vi "Tx.vi"() -> ()   [LabVIEW 2025]
uses:
  <vilib>/sound2/lvsound2.llb/Sound File Position.ctl
  <vilib>/addons/Modulation/Analog/support/mod_Set Error Source.vi
  <vilib>/addons/Modulation/Digital/General/MT Generate PSK System Parameters(M).vi
  <vilib>/addons/Modulation/Digital/Support/Common/Validators/mod_Generate Filter Coefficients Validate.vi
  <vilib>/addons/Modulation/Digital/General/subVIs/mod_Generate Filter Coefficients.vi
  <instrlib>/niUSRP/niUSRP Write Tx Data (CDB).vi
  <vilib>/addons/Modulation/niDMT.lvlib
panel:
  out "IQ Rate (actual)":dbl format="%#_6p"
  out "Carrier Frequency (actucal)":dbl=100000.0 format="%#_6p"
  out "Gain":dbl format="%#_6f"
  in  "modulation type":T1(ring)=enum."PSK"
  out "XY Graph 4":T2(graph)
  out "XY Graph 3":cdb[](graph)
  in  "PSK type":u16(ring) items=["normal", "shifted", "offset"]
  in  "M-PSK (4)":i32=8
  in  "differential PSK":enum16{"disable", "enable"}(ring)
  in  "filter parameter":dbl=0.8 format="%.2f"
  out "symbols out":cdb[](array[numeric]) format="%.2f"
  in  "error in":errorcluster
  out "size(s)":i32
  in  "error in (no error)":errorcluster
  out "error out":errorcluster
  in  "stop":bool
  out "BB Modulate":cluster{"t0":dbl, "dt":dbl, "Y":dbl[]}(graph)
  out "input":i16[](graph)
  in  "active antenna":string="TX1"
  in  "carrier frequency":dbl=2400000000.0 format="%#_6p"
  in  "gain":dbl format="%#_6f"
  in  "IQ rate":dbl=200000.0 format="%#_6p"
  in  "channel list":string
  in  "device names":refnum<k15>="NI2900"
  in  "filter length (symbols)":i32=8
  in  "symbol rate (Hz)":dbl=127500.0 format="%.2f"
  in  "samples per symbol (16)":i32=16
  in  "pulse shaping samples per symbol (16)":i32=16
  in  "pulse shaping filter (none)":T3(ring)=enum."Root Raised Cos"
  in  "number of samples/ch (-1: all)":i32=-1
  in  "start path":path=path ""
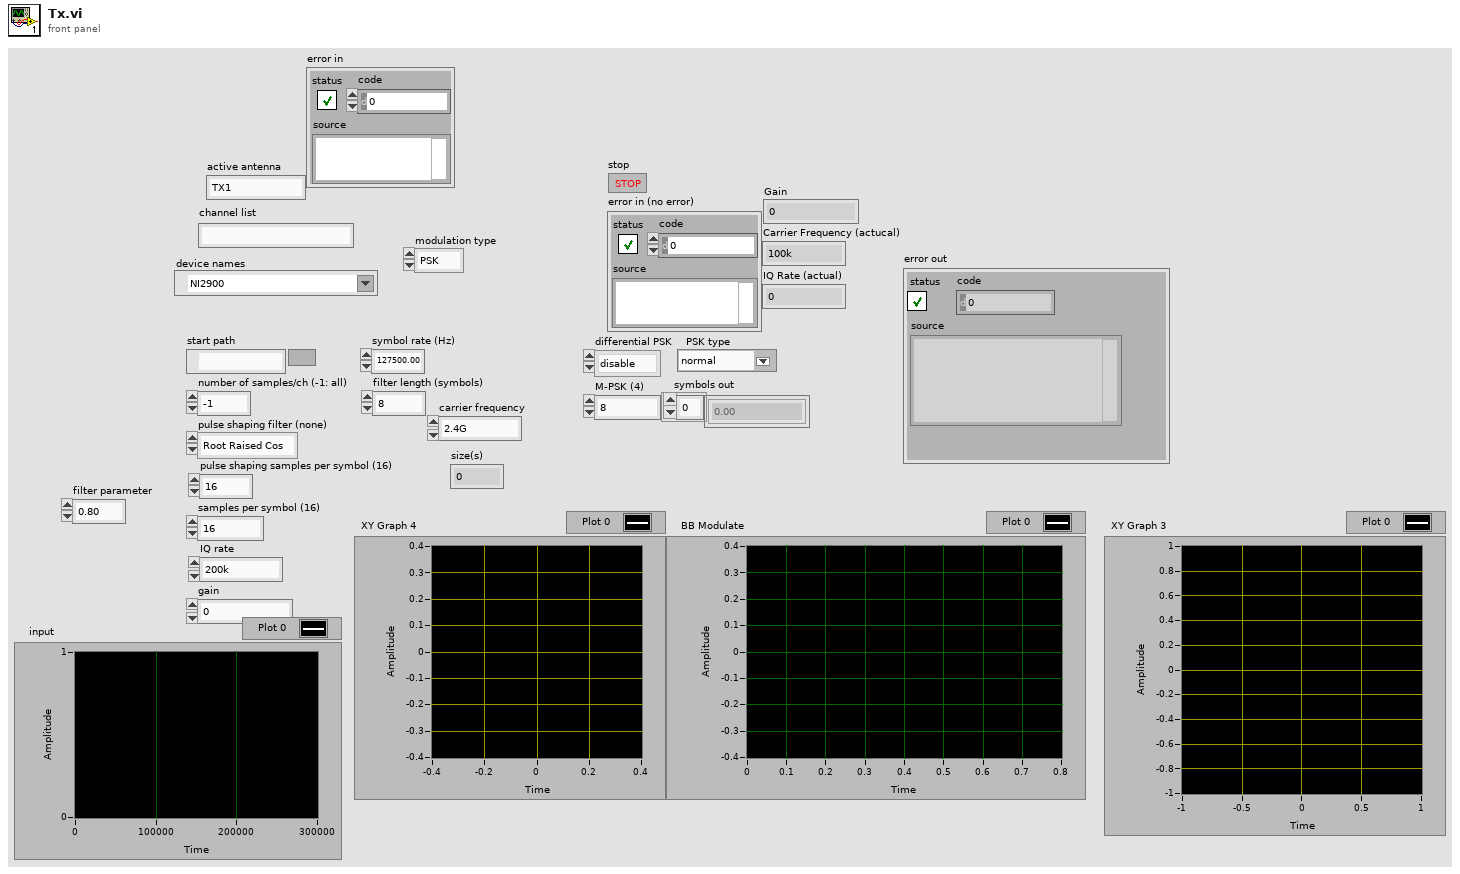
[diagram p1: front panel]
types:
  T1 = enum16{"FSK", "PSK", "QAM", "MSK", "PAM", "ASK", "CPM"}
  T2 = cluster{"constellation":dbl[], "oversampled data":dbl[]}[]
  T3 = enum16{"none", "Raised Cosine", "Root Raised Cos", "Gaussian"}
  T4 = typedef "Sound File Position.ctl" = u16
  T5 = cluster{"samples per symbol (16)":i32, "symbol map":cdb[], "differential PSK":enum16{"disable", "enable"}, "PSK type":u16}
  T6 = typedef "niAMT.lvlib/Complex Data Waveform.ctl" = cluster{"t0":dbl, "dt":dbl, "Y":cdb[]}
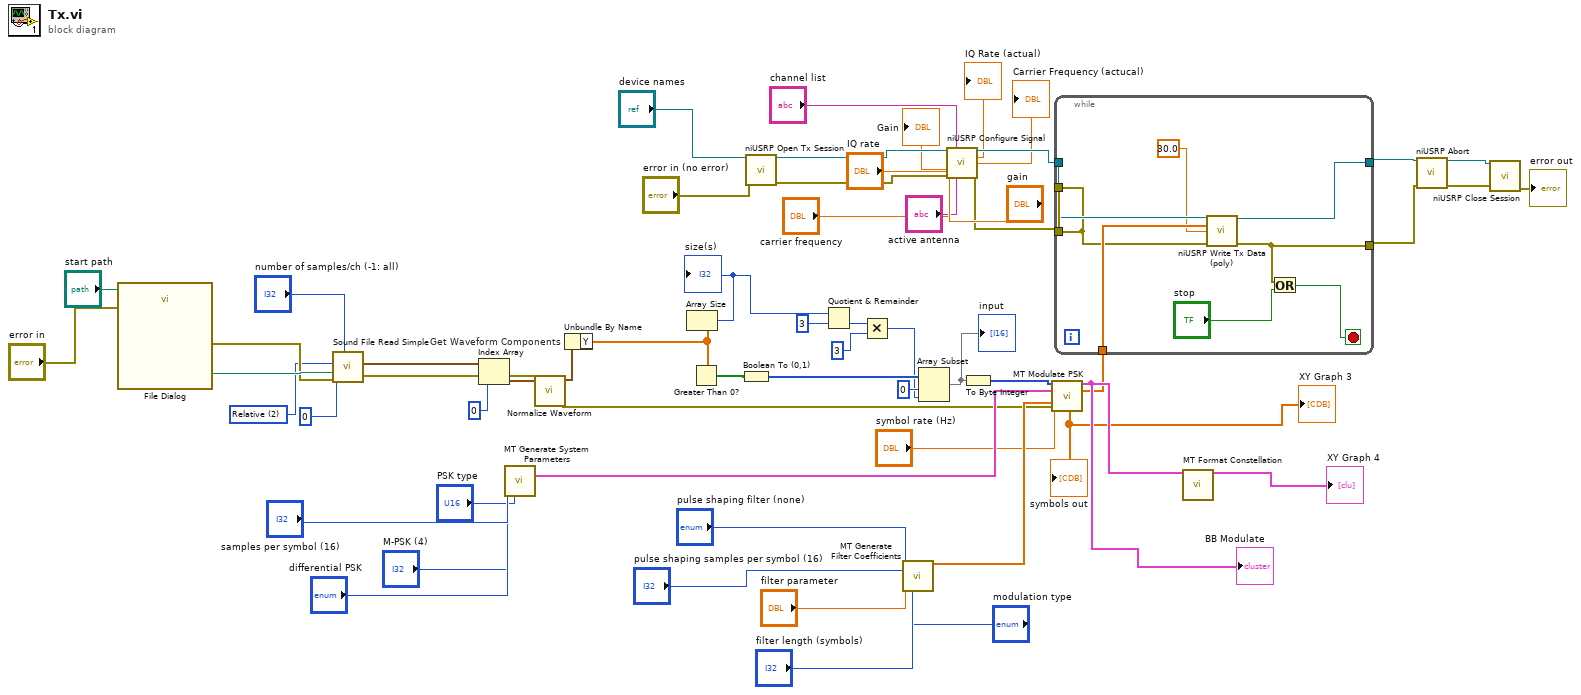
[diagram p0: block diagram]
diagram:
  w14 = T4 2 items=["Absolute"=0, "Relative"=2] ("position mode")
  n1 = call "File Dialog"("start path"="start path", "error in"="error in") -> ("selected path"=w57:path, "error out"=w27:errorcluster)  [unwired: 10 in, 2 out]
  n2 = call <vilib>:"Sound File Read Simple.vi"("number of samples/ch (-1: all)"="number of samples/ch (-1: all)", "error in (no error)"=w27, "position offset"=0, "position mode"=w14, "path"=w57) -> ("error out"=w26:errorcluster, "data"=w56:waveform(dbl)[])  [unwired: 3 in, 2 out]
  n3 = Index Array "Index Array"(array=w56, index=0) -> (element=w52:waveform(dbl))
  n4 = call-poly <vilib>:"MT Generate System Parameters.vi"("samples per symbol (16)"="samples per symbol (16)", "PSK type"="PSK type", "M-PSK (4)"="M-PSK (4)", "differential PSK"="differential PSK") -> ("PSK system parameters"=w40:T5)  [unwired: 9 in, 2 out]
  n5 = call <vilib>:"Normalize Waveform.vi"("error in (no error)"=w26, "waveform in"=w52) -> ("error out"=w25:errorcluster, "normalized waveform"=w51:waveform(dbl))  [unwired: 6 in, 2 out]
  n6 = Unbundle By Name "Get Waveform Components"(w51) -> ("Y"=w48:dbl[])
  n7 = Array Size(array=w48) -> (size(s)=w47:i32)
  "size(s)" <- w47
  n8 = Greater Than 0?(x=w48) -> (x > 0?=w50:bool[])
  n9 = Boolean To (0,1)(Boolean=w50) -> (0, 1=w49:i16[])
  n10 = call <instrlib>:"niUSRP Open Tx Session.vi"("device names"="device names", "error in (no error)"="error in (no error)") -> ("session handle out"=w37:refnum<k15>, "error out"=w24:errorcluster)  [unwired: 12 in]
  n11 = Quotient & Remainder(x=w47, y=3) -> (floor(x/y)=w13:i32)  [unwired: 1 out]
  n12 = Multiply(x=w13, y=3) -> (x*y=w45:i32)
  n13 = call <vilib>:"MT Generate Filter Coefficients.vi"("pulse shaping filter (none)"="pulse shaping filter (none)", "modulation type"="modulation type", "pulse shaping samples per symbol (16)"="pulse shaping samples per symbol (16)", "filter parameter"="filter parameter", "filter length (symbols)"="filter length (symbols)") -> ("pulse shaping filter coefficients"=w42:dbl[])  [unwired: 8 in, 2 out]
  n14 = Array Subset "Array Subset"(array=w49, index=0, length=w45) -> (w2:i16[])
  "input" <- w2
  n15 = call <instrlib>:"niUSRP Configure Signal.vi"("session handle"=w37, "channel list"="channel list", "IQ rate"="IQ rate", "carrier frequency"="carrier frequency", "gain"="gain", "error in (no error)"=w24, "active antenna"="active antenna") -> ("session handle out"=w16:refnum<k15>, "coerced IQ rate"=→"IQ Rate (actual)":dbl, "coerced carrier frequency"=→"Carrier Frequency (actucal)":dbl, "coerced gain"=→"Gain":dbl, "error out"=w15:errorcluster)  [unwired: 4 in]
  n16 = To Byte Integer(number=w2) -> (8bit integer=w1:i8[])
  n17 = call <vilib>:"MT Modulate PSK.vi"("input bit stream"=w1, "PSK system parameters"=w40, "symbol rate (Hz)"="symbol rate (Hz)", "pulse shaping filter coefficients"=w42, "error in (no error)"=w25) -> ("output complex waveform"=w28:T6, "symbols out"=w6:cdb[])  [unwired: 8 in, 1 out]
  "BB Modulate" <- w28
  "symbols out" <- w6
  "XY Graph 3" <- w6
  n18 = while {
    tunnel: [w66] -> w30
    tunnel: [w63] -> w23
    tunnel: w16 -> [w62]
    tunnel: w15 -> [w60]
    tunnel: w6 -> [w61]
    tunnel: [w60] -> _
    stop <- w64 stop-if-true
    n19 = call-poly <instrlib>:"niUSRP Write Tx Data (poly).vi"("session handle"=w62, "data"=w61, "timeout"=30.0, "error in (no error)"=w60) -> ("session handle out"=w66:refnum<k15>, "error out"=w63:errorcluster)  [unwired: 10 in]
    n20 = Or(x=w63, y="stop") -> (x .or. y?=w64:bool)
  }
  n21 = call <vilib>:"MT Format Constellation.vi"("waveform"=w28) -> ("constellation graph"=→"XY Graph 4":T2)  [unwired: 13 in, 1 out]
  n22 = call <instrlib>:"niUSRP Abort.vi"("session handle"=w30, "error in (no error)"=w23) -> ("session handle out"=w29:refnum<k15>, "error out"=w22:errorcluster)  [unwired: 12 in]
  n23 = call <instrlib>:"niUSRP Close Session.vi"("session handle"=w29, "error in (no error)"=w22) -> ("error out"=→"error out":errorcluster)  [unwired: 13 in]
